vi "DllTest.vi"() -> ()   [LabVIEW 2023]
uses:
  D:/Projects/S7View/S7Lib/bin/Debug/S7Lib.dll
  S7Lib/bin/Debug/S7Lib.dll
panel:
  in  "count 3":u16
  in  "value":string
  out "Byte":u8
  in  "bit 2":u8
  in  "start 6":u16
  out "IsRunning":bool
  in  "trim":bool
  out "字符":string="|"
  in  "size 3":u16=20
  in  "start 5":u16=42
  in  "start 4":u16
  in  "count 2":u16
  in  "Bits":bool[](array[boolean])
  in  "bit":u8
  in  "count":u16
  out "字符":string="|"
  in  "size 2":u16=20
  in  "start 3":u16=40
  in  "start 2":u16=62
  in  "size":u16=20
  out "字符串":string="|"
  out "R_DB_Floats":sgl[](array[numeric])
  in  "start":u16
  in  "db":u16=6000
  out "错误输出":errorcluster
  in  "布尔":bool
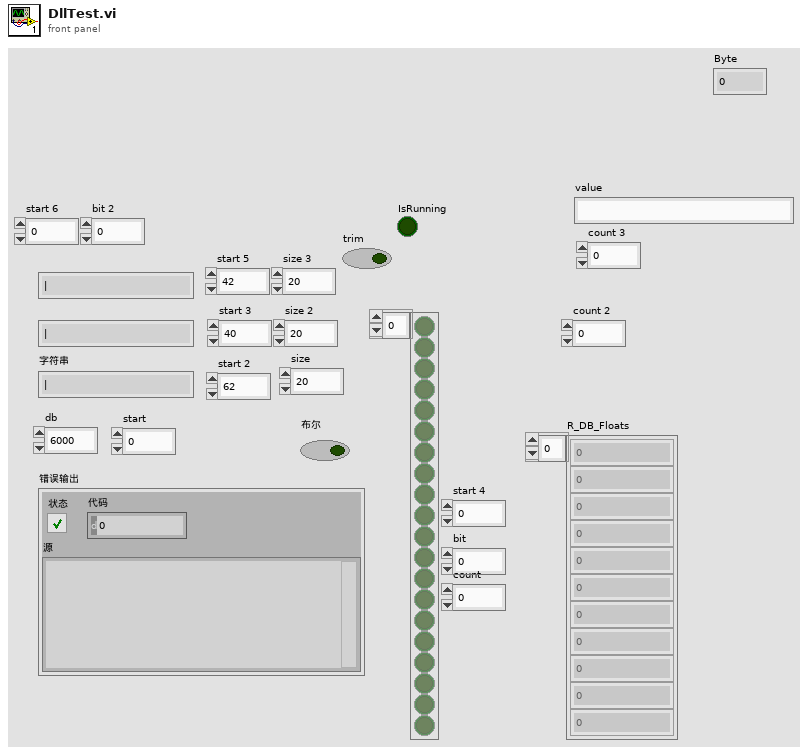
[diagram p1: front panel]
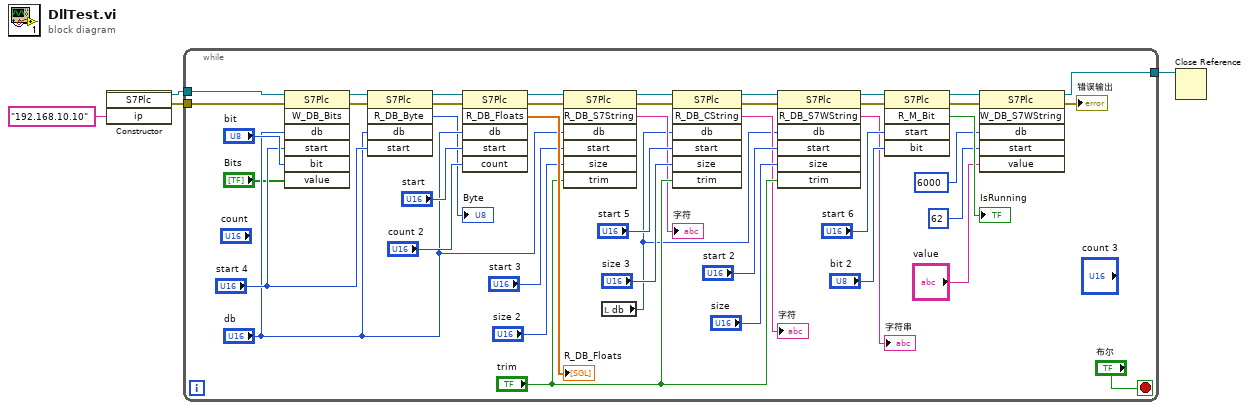
[diagram p0: block diagram]
diagram:
  n1 = constructor class="S7Plc"("ip"="192.168.10.10") -> (reference out=w4:refnum<k24>, error out=w3:errorcluster)  [unwired: 3 in, 2 out]
  n2 = while {
    tunnel: w4 -> [w24]
    tunnel: w3 -> [w48]
    tunnel: [w12] -> w1
    stop <- "布尔" stop-if-true
    n3 = invoke on="调用节点" class="S7Plc" method="W_DB_Bits"(reference=w24, error in=w48, "db"="db", "start"="start 4", "bit"="bit", "value"="Bits") -> (reference out=w33:refnum<k24>, error out=w35:errorcluster)  [unwired: 1 in, 5 out]
    n4 = invoke on="调用节点" class="S7Plc" method="R_DB_Byte"(reference=w33, error in=w35, "db"="db", "start"="start 4") -> (reference out=w32:refnum<k24>, error out=w34:errorcluster, "R_DB_Byte"=→"Byte":u8)  [unwired: 1 in, 2 out]
    n5 = invoke on="调用节点" class="S7Plc" method="R_DB_Floats"(reference=w32, error in=w34, "db"="db", "start"="start", "count"="count 2") -> (reference out=w42:refnum<k24>, error out=w41:errorcluster, "R_DB_Floats"=→"R_DB_Floats":sgl[])  [unwired: 1 in, 3 out]
    n6 = invoke on="调用节点" class="S7Plc" method="R_DB_S7String"(reference=w42, error in=w41, "db"="db", "start"="start 3", "size"="size 2", "trim"="trim") -> (reference out=w27:refnum<k24>, error out=w29:errorcluster, "R_DB_S7String"=→"字符":string)  [unwired: 1 in, 4 out]
    n7 = local read "db"() -> (w14:u16)
    n8 = invoke on="调用节点" class="S7Plc" method="R_DB_CString"(reference=w27, error in=w29, "db"=w14, "start"="start 5", "size"="size 3", "trim"="trim") -> (reference out=w26:refnum<k24>, error out=w28:errorcluster, "R_DB_CString"=→"字符":string)  [unwired: 1 in, 4 out]
    n9 = invoke on="调用节点" class="S7Plc" method="R_DB_S7WString"(reference=w26, error in=w28, "db"=w14, "start"="start 2", "size"="size", "trim"="trim") -> (reference out=w20:refnum<k24>, error out=w19:errorcluster, "R_DB_S7WString"=→"字符串":string)  [unwired: 1 in, 4 out]
    n10 = invoke on="调用节点" class="S7Plc" method="R_M_Bit"(reference=w20, error in=w19, "start"="start 6", "bit"="bit 2") -> (reference out=w8:refnum<k24>, error out=w7:errorcluster, "R_M_Bit"=→"IsRunning":bool)  [unwired: 1 in, 2 out]
    n11 = invoke on="调用节点" class="S7Plc" method="W_DB_S7WString"(reference=w8, error in=w7, "db"=u16 6000, "start"=u16 62, "value"="value") -> (reference out=w12:refnum<k24>, error out=→"错误输出":errorcluster)  [unwired: 1 in, 4 out]
  }
  n12 = Close Reference(reference=w1) -> ()  [unwired: 1 in, 1 out]
